vi "TDMS_Finalize.vi"(8 "error in (no error)":errorcluster, 11 "state in":T1={"ref TDMS"=refnum, "File Path"=path "", "counter"=0, "Folder tmp"=path "/home/lvuser/lab9data/tmp", "folder ready"=path "/home/lvuser/lab9data/ready"}) -> (0 "error out":errorcluster)   [LabVIEW 2025]
uses:
  Logger_State.ctl
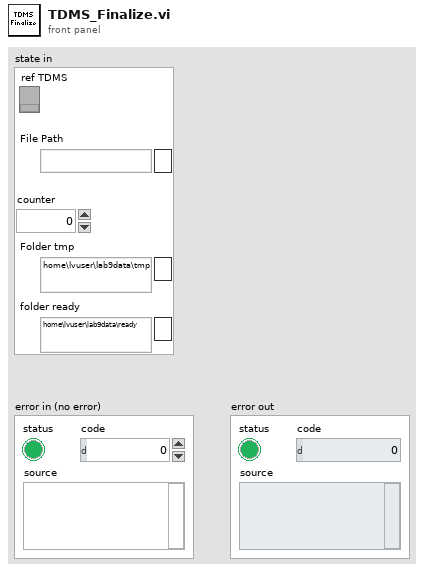
[diagram p1: front panel]
types:
  T1 = typedef "Logger_State.ctl" = cluster{"ref TDMS":refnum<k34>, "File Path":path, "counter":i32, "Folder tmp":path, "folder ready":path}
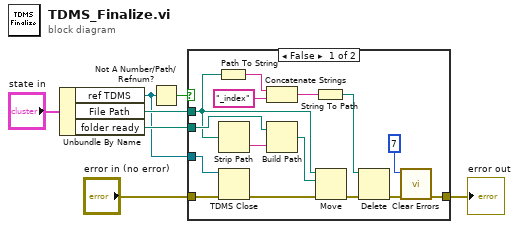
[diagram p0: block diagram]
diagram:
  n1 = Unbundle By Name("state in") -> ("ref TDMS"=w4:refnum<k34>, "File Path"=w5:path, "folder ready"=w6:path)
  n2 = Not A Number/Path/Refnum?(number/path/refnum=w4) -> (NaN/Path/Refnum?=w2:bool)
  n3 = case shown="False" w2 {
    tunnel: "error in (no error)" -> [w22 w23]
    tunnel: w4 -> [w21 _]
    tunnel: w5 -> [w16 _]
    tunnel: w6 -> [w19 _]
    tunnel: [w9 w23] -> w7
    frame False {
      n4 = Path To String(path=w16) -> (string=w15:string)
      n5 = Strip Path(path=w16) -> (name=w20:string)  [unwired: 1 out]
      n6 = TDMS Close(8:w22, 11:w21) -> (0:w17:errorcluster)  [unwired: 1 out]
      n7 = Concatenate Strings(w15, "_index" ("string")) -> (w13:string)
      n8 = Build Path(base path=w19, name or relative path=w20) -> (appended path=w18:path)
      n9 = String To Path(string=w13) -> (path=w12:path)
      n10 = Move(source path=w16, error in=w17, 10:w18) -> (error out=w11:errorcluster)  [unwired: 2 in, 2 out]
      n11 = Delete(path (use dialog)=w12, error in=w11) -> (error out=w10:errorcluster)  [unwired: 3 in, 2 out]
      n12 = call <vilib>:"Clear Errors.vi"("error in (no error)"=w10, "specific error code to clear (0: all)"=7) -> ("error out"=w9:errorcluster)  [unwired: 4 in, 1 out]
    }
    frame True {
    }
  }
  "error out" <- w7
